vi "test open previous test (1).vi"() -> ()   [LabVIEW 2019]
panel:
  out "error out 2":errorcluster
  out "standard output 2":string
  out "standard error 2":string
  in  "Open":bool
  out "standard error":string
  out "standard output":string
  out "error out":errorcluster
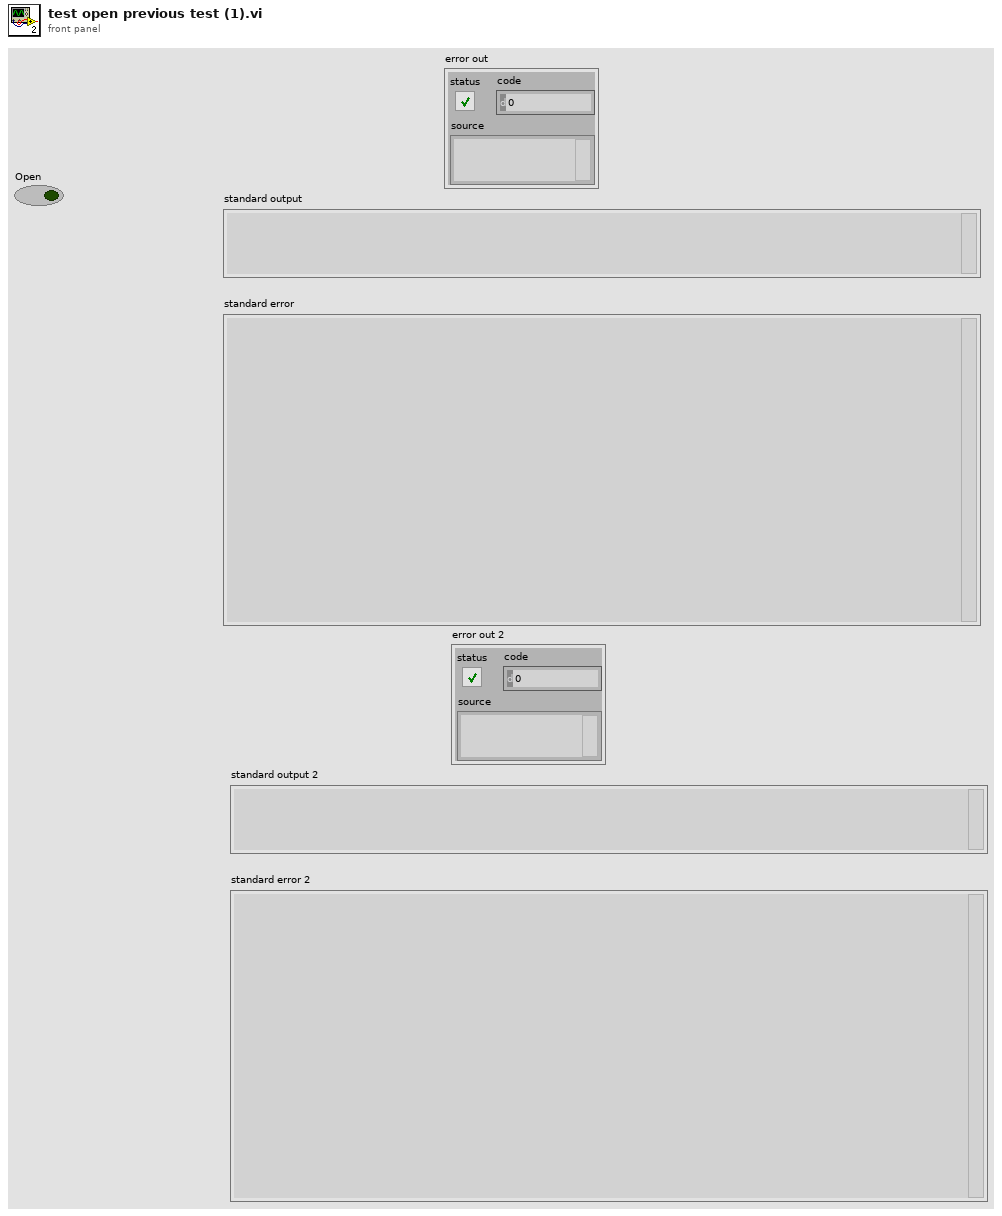
[diagram p1: front panel]
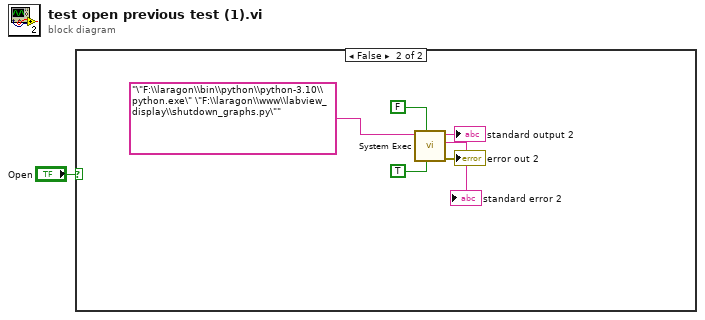
[diagram p0: block diagram]
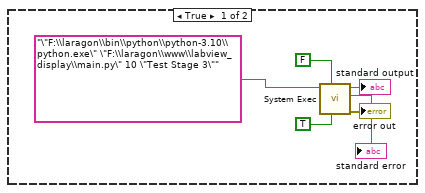
[diagram p2: hidden frame]
diagram:
  n1 = case shown="False" "Open" {
    frame True {
      n2 = call <vilib>:"System Exec.vi"("run minimized? (F)"=TRUE, "wait until completion? (T)"=FALSE, "command line"="\"F:\\laragon\\bin\\python\\python-3.10\\python.exe\" \"F:\\laragon\\www\\labview_display\\main.py\" 10 \"Test Stage 3\"") -> ("error out"=→"error out":errorcluster, "standard error"=→"standard error":string, "standard output"=→"standard output":string)  [unwired: 5 in, 1 out]
    }
    frame False {
      n3 = call <vilib>:"System Exec.vi"("run minimized? (F)"=TRUE, "wait until completion? (T)"=FALSE, "command line"="\"F:\\laragon\\bin\\python\\python-3.10\\python.exe\" \"F:\\laragon\\www\\labview_display\\shutdown_graphs.py\"") -> ("error out"=→"error out 2":errorcluster, "standard error"=→"standard error 2":string, "standard output"=→"standard output 2":string)  [unwired: 5 in, 1 out]
    }
  }
